vi "Local_write.vi"(9 "内容":string, 10 "名字":string) -> (2 "错误输出":errorcluster)   [LabVIEW 2018, in "Log_class.lvlib"]
uses:
  Log_class.lvlib
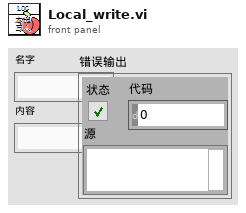
[diagram p1: front panel]
types:
  T1 = enum16{"open", "replace", "create", "open or create", "replace or create", "replace or create with confirmation"}
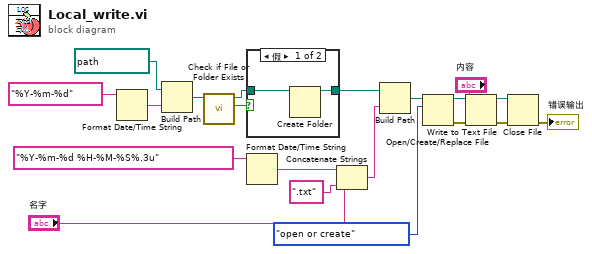
[diagram p0: block diagram]
diagram:
  n1 = Format Date/Time String(time format string (%c)="%Y-%m-%d" ("时间格式字符串(%c)")) -> (date/time string=w4:string)  [unwired: 2 in]
  n2 = Build Path(base path=path "D:/日志" ("文件路径（使用对话框）"), name or relative path=w4) -> (appended path=w11:path)
  n3 = call <vilib>:"Check if File or Folder Exists.vi"("path"=w11) -> ("file or folder exists?"=w10:bool, "dup path"=w9:path)  [unwired: 8 in, 1 out]
  n4 = case shown="假" w10 {
    tunnel: w9 -> [w22 w23]
    tunnel: [w21 w23] -> w8
    frame False {
      n5 = Create Folder(path (use dialog)=w22) -> (created path=w21:path)  [unwired: 2 in, 2 out]
    }
    frame True {
    }
  }
  n6 = Format Date/Time String(time format string (%c)="%Y-%m-%d %H-%M-%S%.3u" ("时间格式字符串(%c)")) -> (date/time string=w6:string)  [unwired: 2 in]
  n7 = Concatenate Strings(w6, "名字", ".txt" ("字符串")) -> (w19:string)
  n8 = Build Path(base path=w8, name or relative path=w19) -> (appended path=w17:path)
  n9 = Open/Create/Replace File(file path (use dialog)=w17, operation (0:open)=T1."open or create" ("操作(0:open)")) -> (refnum out=w16:refnum<file>, error out=w15:errorcluster)  [unwired: 4 in, 1 out]
  n10 = Write to Text File(file (use dialog)=w16, text="内容", error in=w15) -> (refnum out=w14:refnum<file>, error out=w13:errorcluster)  [unwired: 1 in, 1 out]
  n11 = Close File(refnum=w14, error in=w13) -> (error out=→"错误输出":errorcluster)  [unwired: 1 out]
